vi "UNITTEST-JSON-RPC-Error-Object.vi"(8 "error in (no error)":errorcluster) -> (0 "error out":errorcluster)   [LabVIEW 2019]
uses:
  <vilib>/addons/_JKI Toolkits/Caraya/classes/Assert/Assert Not Error.vi
  <vilib>/addons/_JKI Toolkits/Caraya/classes/Assert/Assert False.vi
  <vilib>/addons/_JKI Toolkits/Caraya/classes/Assert/Assert True.vi
  JSON-RPC/JSON-RPC.lvlib
  <vilib>/addons/_JKI Toolkits/Caraya/classes/Assert/Assert.lvclass
  <vilib>/addons/_JKI Toolkits/Caraya/classes/Test/Test.lvclass
  <vilib>/JDP Science/JSONtext/JSONtext.lvlib
panel:
  out "Array":string[](array[string])
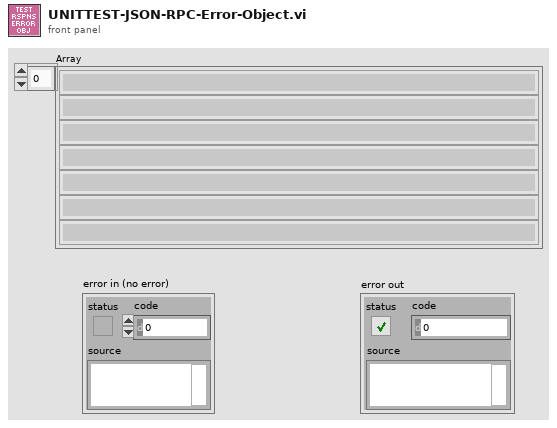
[diagram p1: front panel]
types:
  T1 = cluster{"error in (no error)":errorcluster, "id":string, "response":string}[]
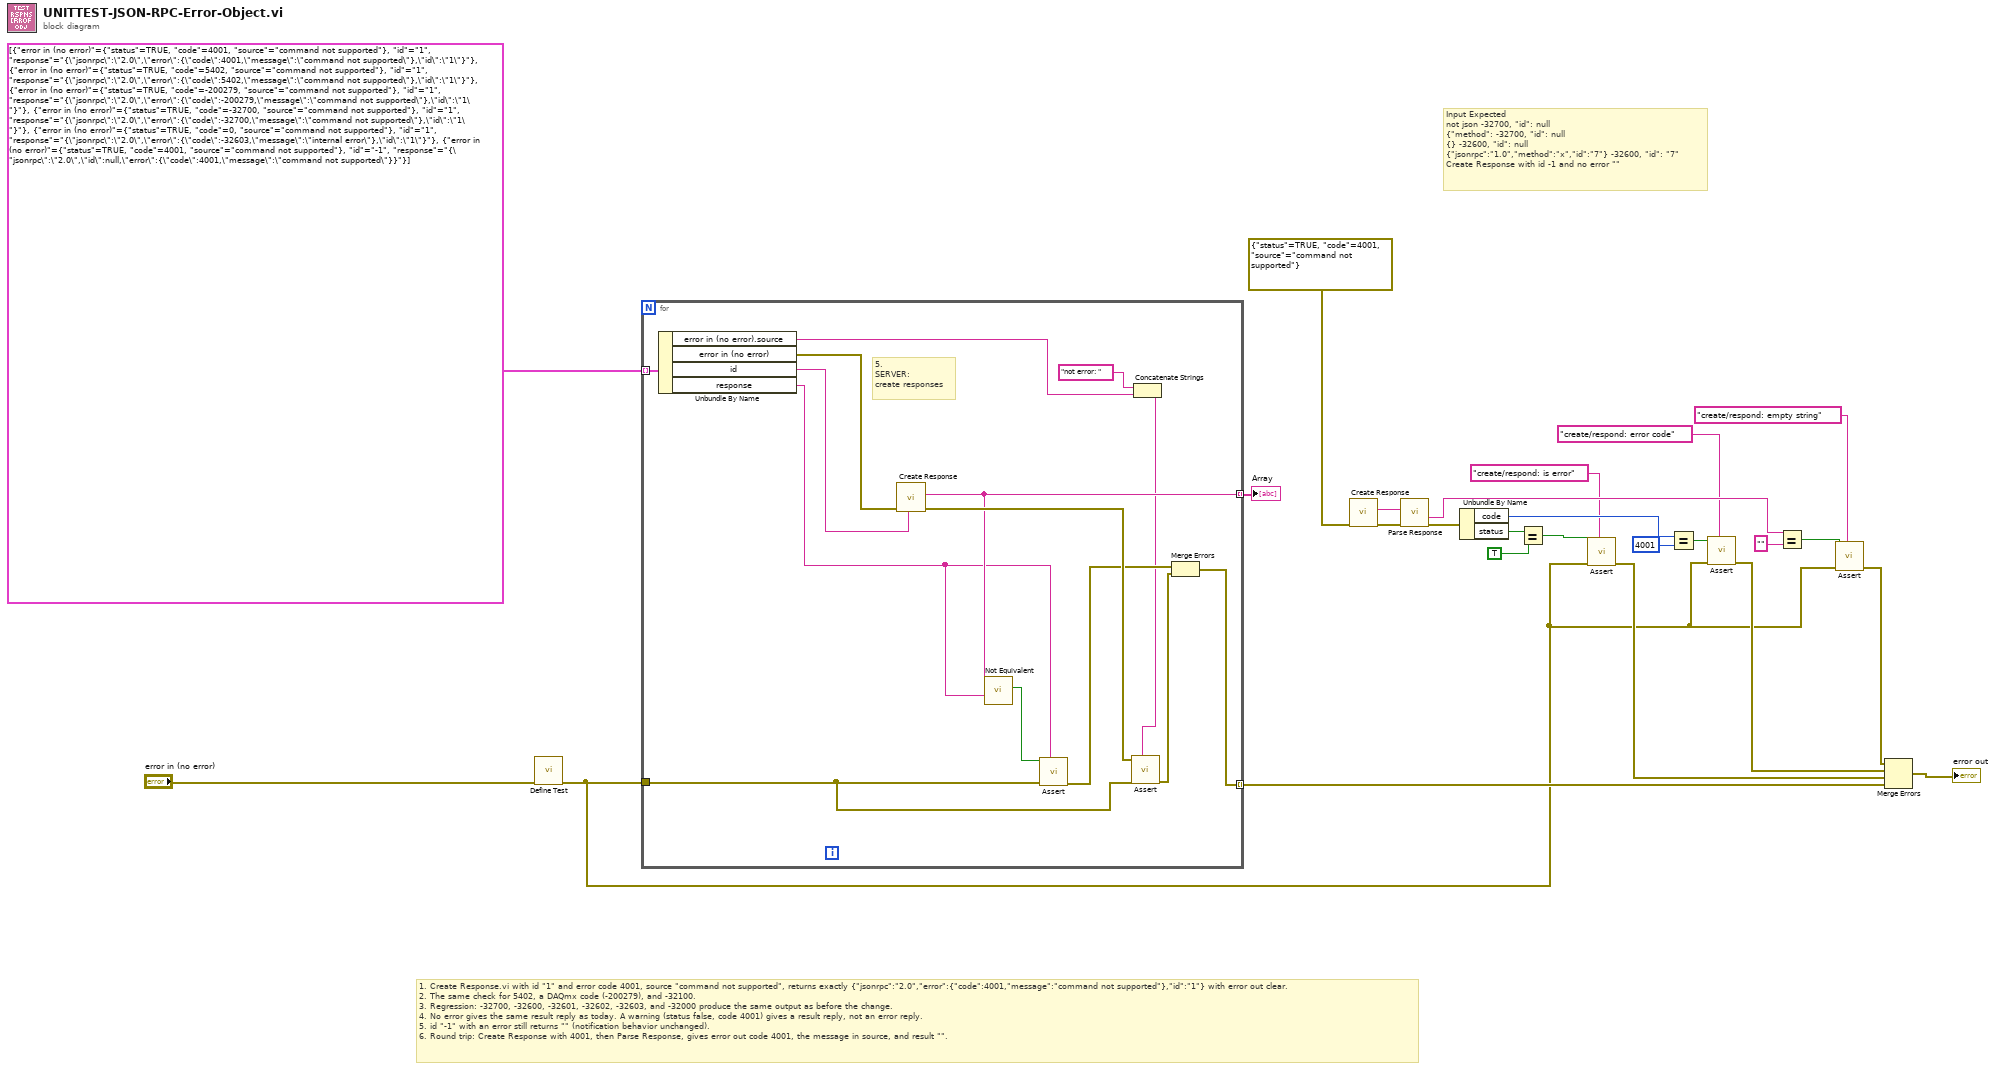
[diagram p0: block diagram]
diagram:
  # "Input\tExpected\nnot json\t-32700, \"id\": null\n{\"method\":\t-32700, \"id\": null\n{}\t-32600, \"id\": null\n{\"jsonrpc\":\"1.0\",\"method\":\"x\",\"id\":\"7\"}\t-32600, \"id\": \"7\"\nCreate Response with id -1 and no error\t\"\""
  # "1. Create Response.vi with id \"1\" and error code 4001, source \"command not supported\", returns exactly {\"jsonrpc\":\"2.0\",\"error\":{\"code\":4001,\"message\":\"command not supported\"},\"id\":\"1\"} with error out clear.\n2. The same check for 5402, a DAQmx code (-200279), and -32100.\n3. Regression: -32700, -32600, -32601, -32602, -32603, and -32000 produce the same output as before the change.\n4. No error gives the same result reply as today. A warning (status false, code 4001) gives a result reply, not an error reply.\n5. id \"-1\" with an error still returns \"\" (notification behavior unchanged).\n6. Round trip: Create Response with 4001, then Parse Response, gives error out code 4001, the message in source, and result \"\"."
  n1 = call <vilib>:"Define Test.vi"("error in (no error)"="error in (no error)") -> ("error out"=w1:errorcluster)  [unwired: 9 in, 1 out]
  n2 = for {
    tunnel: [w31] -> w24 mode=indexing
    tunnel: w1 -> [w38]
    tunnel: [w35] -> w5 mode=indexing
    tunnel: T1 [{"error in (no error)"={"status"=TRUE, "code"=4001, "source"="command not supported"}, "id"="1", "response"="{\"jsonrpc\":\"2.0\",\"error\":{\"code\":4001,\"message\":\"command not supported\"},\"id\":\"1\"}"}, {"error in (no error)"={"status"=TRUE, "code"=5402, "source"="command not supported"}, "id"="1", "response"="{\"jsonrpc\":\"2.0\",\"error\":{\"code\":5402,\"message\":\"command not supported\"},\"id\":\"1\"}"}, {"error in (no error)"={"status"=TRUE, "code"=-200279, "source"="command not supported"}, "id"="1", "response"="{\"jsonrpc\":\"2.0\",\"error\":{\"code\":-200279,\"message\":\"command not supported\"},\"id\":\"1\"}"}, {"error in (no error)"={"status"=TRUE, "code"=-32700, "source"="command not supported"}, "id"="1", "response"="{\"jsonrpc\":\"2.0\",\"error\":{\"code\":-32700,\"message\":\"command not supported\"},\"id\":\"1\"}"}, {"error in (no error)"={"status"=TRUE, "code"=0, "source"="command not supported"}, "id"="1", "response"="{\"jsonrpc\":\"2.0\",\"error\":{\"code\":-32603,\"message\":\"internal error\"},\"id\":\"1\"}"}, {"error in (no error)"={"status"=TRUE, "code"=4001, "source"="command not supported"}, "id"="-1", "response"="{\"jsonrpc\":\"2.0\",\"id\":null,\"error\":{\"code\":4001,\"message\":\"command not supported\"}}"}] -> [w34] mode=indexing
    # "5.\nSERVER:\ncreate responses"
    n3 = Unbundle By Name(w34) -> ("error in (no error).source"=w27:string, "error in (no error)"=w33:errorcluster, "id"=w32:string, "response"=w29:string)
    n4 = call "Create Response.vi"("id"=w32, "error in (no error)"=w33) -> ("error out"=w39:errorcluster, "<JSON> Response"=w31:string)  [unwired: 8 in]
    n5 = call <vilib>:"Not Equivalent.vi"("Other JSON"=w29, "JSON"=w31) -> ("Not Equivalent"=w30:bool)  [unwired: 8 in]
    n6 = call-poly <vilib>:"Assert.vi"("Label"=w29, "error in (no error)"=w38, "False?"=w30) -> ("error out"=w37:errorcluster)  [unwired: 7 in, 1 out]
    n7 = Concatenate Strings("not error: ", w27) -> (w26:string)
    n8 = call-poly <vilib>:"Assert.vi"("Label"=w26, "error in (no error)"=w38, "Not Error?"=w39) -> ("error out"=w36:errorcluster)  [unwired: 7 in, 1 out]
    n9 = Merge Errors(w37, w36) -> (w35:errorcluster)
  }
  "Array" <- w24
  n10 = call "Create Response.vi"("error in (no error)"=errorcluster {"status"=TRUE, "code"=4001, "source"="command not supported"}) -> ("error out"=w22:errorcluster, "<JSON> Response"=w21:string)  [unwired: 9 in]
  n11 = call "Parse Response.vi"("error in (no error)"=w22, "<JSON> Response"=w21) -> ("error out"=w20:errorcluster, "results"=w13:string)  [unwired: 7 in, 1 out]
  n12 = Unbundle By Name(w20) -> ("code"=w15:i32, "status"=w19:bool)
  n13 = Equal?(x=w19, y=TRUE) -> (x = y?=w17:bool)
  n14 = call-poly <vilib>:"Assert.vi"("Label"="create/respond: is error", "error in (no error)"=w1, "True?"=w17) -> ("error out"=w8:errorcluster)  [unwired: 7 in, 1 out]
  n15 = Equal?(x=w15, y=4001) -> (x = y?=w16:bool)
  n16 = call-poly <vilib>:"Assert.vi"("Label"="create/respond: error code", "error in (no error)"=w1, "True?"=w16) -> ("error out"=w9:errorcluster)  [unwired: 7 in, 1 out]
  n17 = Equal?(x=w13, y="") -> (x = y?=w11:bool)
  n18 = call-poly <vilib>:"Assert.vi"("Label"="create/respond: empty string", "error in (no error)"=w1, "True?"=w11) -> ("error out"=w10:errorcluster)  [unwired: 7 in, 1 out]
  n19 = Merge Errors(w10, w9, w8, w5) -> (→"error out":errorcluster)
